vi "CIVI Read Frequency Example.vi"() -> ()   [LabVIEW 2026]
panel:
  out "S Meter out":errorcluster
  out "S Meter":i32
  out "Mode error out":errorcluster
  out "Mode":string
  out "error out":errorcluster
  out "Frequency (Hz)":i32
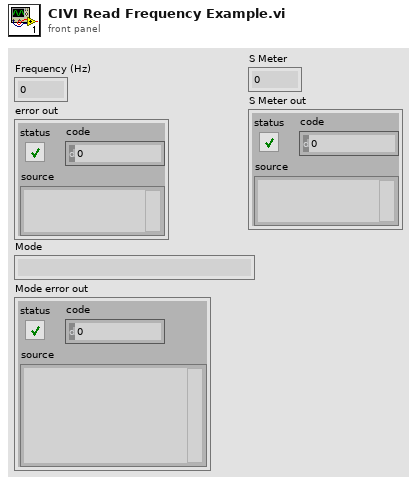
[diagram p1: front panel]
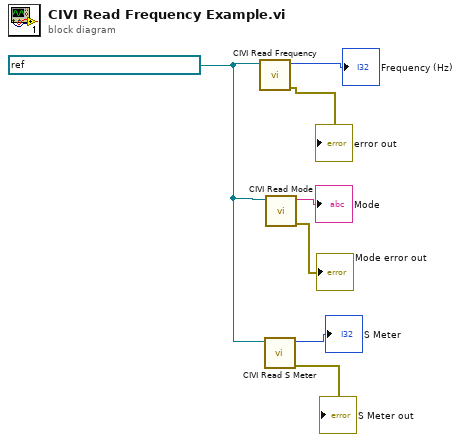
[diagram p0: block diagram]
diagram:
  w1 = refnum<visa-resource-name> "TCPIP0::127.0.0.1::5025::SOCKET" ("VISA Resource Name")
  n1 = call "CIVI Read Frequency.vi"("VISA Resource Name"=w1) -> ("error out"=→"error out":errorcluster, "Frequency (Hz)"=→"Frequency (Hz)":i32)  [unwired: 9 in]
  n2 = call "CIVI Read S Meter.vi"("VISA Resource Name"=w1) -> ("error out"=→"S Meter out":errorcluster, "S Meter (raw)"=→"S Meter":i32)  [unwired: 9 in]
  n3 = call "CIVI Read Mode.vi"("VISA Resource Name"=w1) -> ("error out"=→"Mode error out":errorcluster, "Mode"=→"Mode":string)  [unwired: 9 in]
